vi "[ce] Wait Until Next ms Multiple (dataflow ready).vi"(5 "boolean in":bool, 6 "error in":errorcluster, 8 "Wait if error (F)":bool, 9 "millisecond multiple":u32) -> (0 "error out":errorcluster, 1 "false":bool, 2 "true":bool=TRUE, 3 "millisecond timer value":u32, 4 "dup boolean in":bool)   [LabVIEW 2021]
doc: "The VI waits until the value of the millisecond timer becomes a multiple of the specified <B>millisecond multiple</B>. If <B>error in</B> indicates any error and <B>Wait if error</B> is FALSE, the VI does not wait and returns current value of the millisecond timer.\n\n<B>boolean in</B> has no effect on VI execution, its value is returned in <B>dup boolean in</B> indicator.\n\n<B>false</B> indicator always returns FALSE. <B>true</B> indicator always returns TRUE. \n\n<B>error out</B> indicator returns the same values as <B>error in</B>\n\n::: CalcExpress Toolkit :::\nCopyright (c) 2000-2026 Konstantin Shifershteyn. All rights reserved."
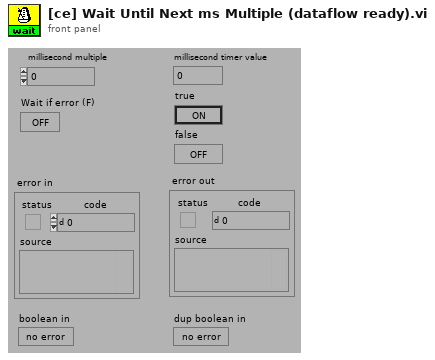
[diagram p1: front panel]
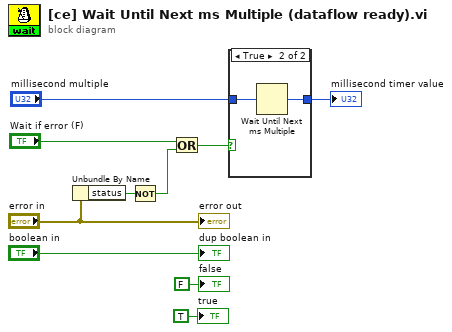
[diagram p0: block diagram]
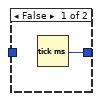
[diagram p2: hidden frame]
diagram:
  n1 = Unbundle By Name("error in") -> ("status"=w6:bool)
  n2 = Not(x=w6) -> (.not. x?=w7:bool)
  n3 = Or(x="Wait if error (F)", y=w7) -> (x .or. y?=w3:bool)
  n4 = case shown="True" w3 {
    tunnel: "millisecond multiple" -> [_ w13]
    tunnel: [w11 w12] -> w8
    frame False {
      n5 = Tick Count (ms)() -> (millisecond timer value=w11:u32)
    }
    frame True {
      n6 = Wait Until Next ms Multiple(millisecond multiple=w13) -> (millisecond timer value=w12:u32)
    }
  }
  "millisecond timer value" <- w8
  "error out" <- "error in"
  "true" <- TRUE ("true")
  "false" <- FALSE ("false")
  "dup boolean in" <- "boolean in"
